vi "Log.vi"(8 "error in":errorcluster, 10 "Log Entry":T1 {"Time" format="%<%x %.3X>T"}, 11 "Mock Logger in":refnum<class "Mock Logger.lvclass">) -> (0 "error out":errorcluster, 3 "Mock Logger out":refnum<class "Mock Logger.lvclass">)   [LabVIEW 2026, in "Mock Logger.lvlib" / "Mock Logger.lvclass"]
doc: "Log the provided entry."
uses:
  Type Definitions/Log Entry--cluster.ctl
  Mock Logger.lvclass
  Mock Logger.lvclass/Mock Logger.ctl
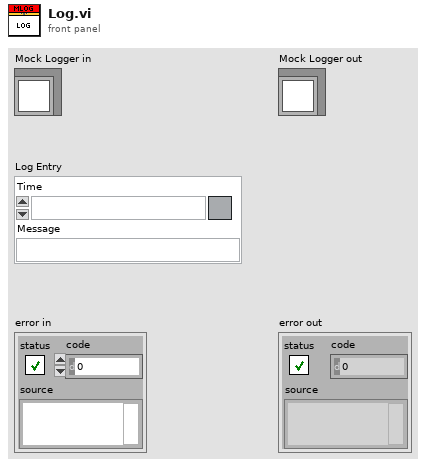
[diagram p1: front panel]
types:
  T1 = typedef "Log Entry--cluster.ctl" = cluster{"Time":timestamp, "Message":string}
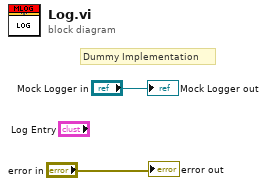
[diagram p0: block diagram]
diagram:
  # "Dummy Implementation"
  "error out" <- "error in"
  "Mock Logger out" <- "Mock Logger in"
